vi "SwerveKinematics_ToSwerveModuleStates.vi"(9 "CenterOfRotation":T3={"X"=0.0, "Y"=1.0} {"Y" format="%14.3f"; "X" format="%14.3f"}, 10 "ChassisSpeeds":T6 {"vOmega" format="%10.3f"; "vY" format="%10.3f"; "vX" format="%10.3f"}, 11 "in SWERVE_DRIVE_KINEMATICS":T4 {"SavedModuleStates"."Angle"."SIN" format="%13.4f"; "SavedModuleStates"."Angle"."COS" format="%13.4f"; "SavedModuleStates"."Angle"."VALUE" format="%13.4f"; "PrevCoR"."Y" format="%14.3f"; "PrevCoR"."X" format="%14.3f"; "Modules"."Y" format="%14.3f"; "Modules"."X" format="%14.3f"}) -> (1 "ModuleStates":T1[](array[typedef]) {"Angle"."SIN" format="%13.4f"; "Angle"."COS" format="%13.4f"; "Angle"."VALUE" format="%13.4f"}, 3 "out SWERVE_DRIVE_KINEMATICS":T4 {"SavedModuleStates"."Angle"."SIN" format="%13.4f"; "SavedModuleStates"."Angle"."COS" format="%13.4f"; "SavedModuleStates"."Angle"."VALUE" format="%13.4f"; "PrevCoR"."Y" format="%14.3f"; "PrevCoR"."X" format="%14.3f"; "Modules"."Y" format="%14.3f"; "Modules"."X" format="%14.3f"})   [LabVIEW 2019, in "Trajectory_Library.lvlib"]
doc: "Performs inverse kinematics to return the module states from a desired chassis velocity. This method is often used to convert joystick values into module speeds and angles.\n \nThis function also supports variable centers of rotation. During normal operations, the center of rotation is usually the same as the physical center of the robot; therefore, the argument is defaulted to that use case. However, if you wish to change the center of rotation for evasive manuevers, vision alignment, or for any other use case, you can do so.\n\nIn the case that the desired chassis speeds are zero (i.e. the robot will be stationary), the previously calculated module angle will be maintained.\n \nParameters:\n - chassisSpeeds -- The desired chassis speed.\n - centerOfRotation -- The center of rotation. For example, if you set the center of rotation at one corner of the robot and provide a chassis speed that only has a dtheta component, the robot will rotate around that corner. (Meters)\n\nReturns:\n - ModuleStates - An array of data structures containing the module states. Use caution because these module states are not normalized. Sometimes, a user input may cause one of the module speeds to go above the attainable max velocity. Use the {@link #normalizeWheelSpeeds(SwerveModuleState[], double) normalizeWheelSpeeds} function to rectify this issue."
uses:
  Trajectory_Library.lvlib
  TypeDef/SWERVE_DRIVE_KINEMATICS.ctl
  <vilib>/Analysis/Matrix/Datatypes/RealMatrix.ctl
  TypeDef/TRANSLATION2D.ctl
  TypeDef/SWERVE_DRIVE_MODULE_STATE.ctl
  TypeDef/ROTATION2D.ctl
  TypeDef/CHASSIS_SPEEDS.ctl
  MatBuilder_Create.vi
  MatrixHelper_CoerceSize.vi
  <vilib>/Analysis/Matrix/Numeric/Multiply/Multiply - RM,RM.vi
  <vilib>/Analysis/Matrix/NI_Matrix.lvlib
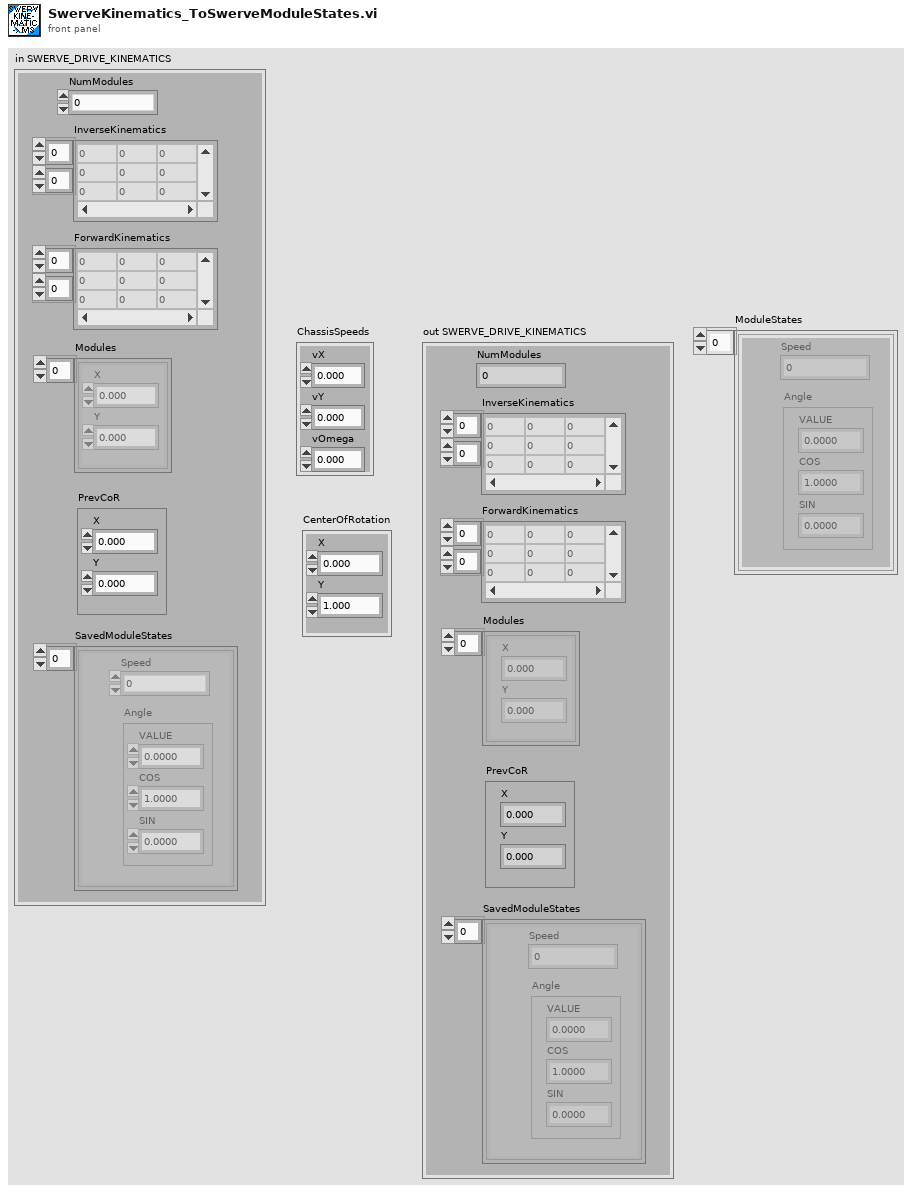
[diagram p1: front panel]
types:
  T1 = typedef "Trajectory_Library.lvlib/SWERVE_DRIVE_MODULE_STATE.ctl" = cluster{"Speed":dbl, "Angle":T2}
  T2 = typedef "Trajectory_Library.lvlib/ROTATION2D.ctl" = cluster{"VALUE":dbl, "COS":dbl, "SIN":dbl}
  T3 = typedef "Trajectory_Library.lvlib/TRANSLATION2D.ctl" = cluster{"X":dbl, "Y":dbl}
  T4 = typedef "Trajectory_Library.lvlib/SWERVE_DRIVE_KINEMATICS.ctl" = cluster{"NumModules":i32, "InverseKinematics":T5, "ForwardKinematics":T5, "Modules":T3[], "PrevCoR":T3, "SavedModuleStates":T1[]}
  T5 = typedef "NI_Matrix.lvlib/RealMatrix.ctl" = dbl[][]
  T6 = typedef "Trajectory_Library.lvlib/CHASSIS_SPEEDS.ctl" = cluster{"vX":dbl, "vY":dbl, "vOmega":dbl}
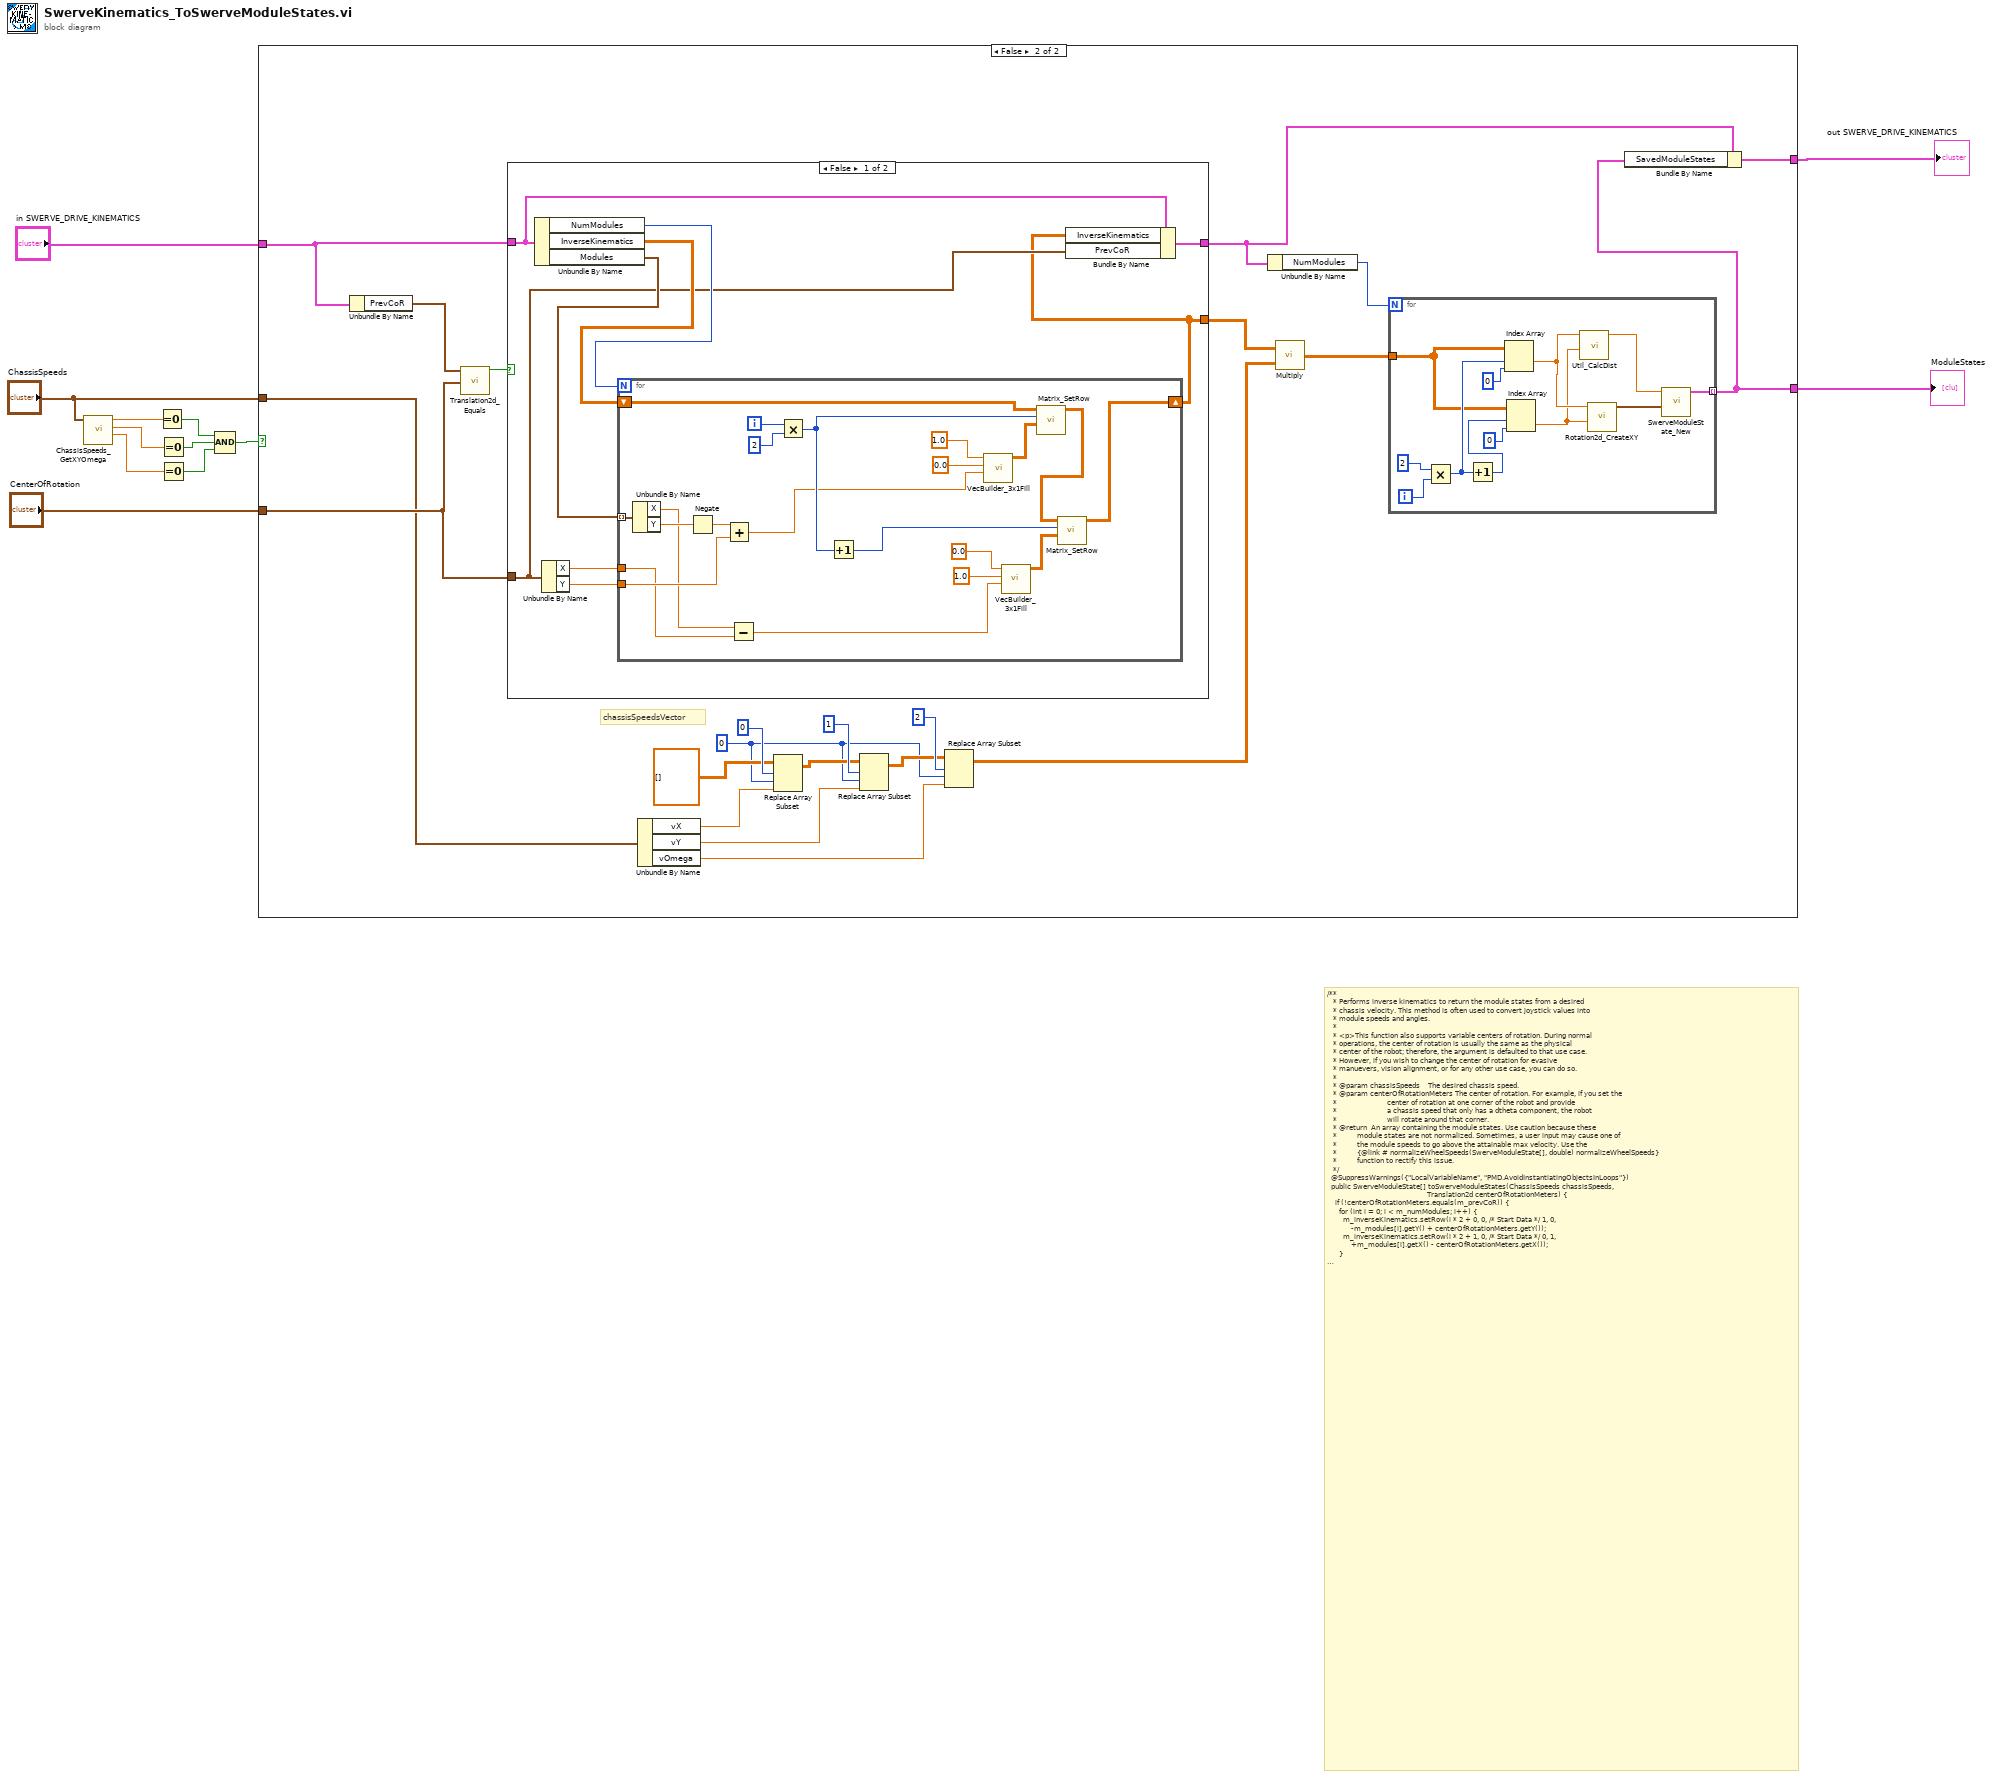
[diagram p0: block diagram]
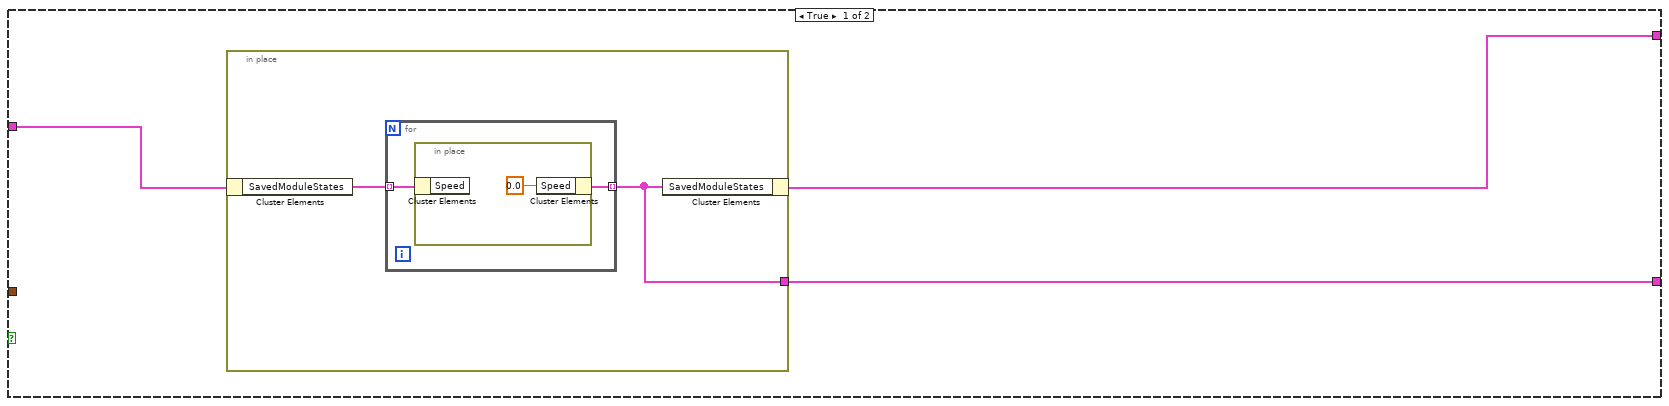
[diagram p2: hidden frame]
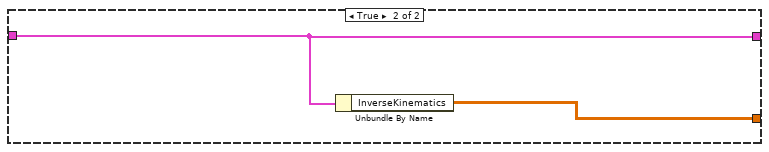
[diagram p3: hidden frame]
diagram:
  # "/**\n   * Performs inverse kinematics to return the module states from a desired\n   * chassis velocity. This method is often used to convert joystick values into\n   * module speeds and angles.\n   *\n   * <p>This function also supports variable centers of rotation. During normal\n   * operations, the center of rotation is usually the same as the physical\n   * center of the robot; therefore, the argument is defaulted to that use case.\n   * However, if you wish to change the center of rotation for evasive\n   * manuevers, vision alignment, or for any other use case, you can do so.\n   *\n   * @param chassisSpeeds    The desired chassis speed.\n   * @param centerOfRotationMeters The center of rotation. For example, if you set the\n   *                         center of rotation at one corner of the robot and provide\n   *                         a chassis speed that only has a dtheta component, the robot\n   *                         will rotate around that corner.\n   * @return  An array containing the module states. Use caution because these\n   *          module states are not normalized. Sometimes, a user input may cause one of\n   *          the module speeds to go above the attainable max velocity. Use the\n   *          {@link # normalizeWheelSpeeds(SwerveModuleState[], double) normalizeWheelSpeeds}\n   *          function to rectify this issue.\n   */\n  @SuppressWarnings({\"LocalVariableName\", \"PMD.AvoidInstantiatingObjectsInLoops\"})\n  public SwerveModuleState[] toSwerveModuleStates(ChassisSpeeds chassisSpeeds,\n                                                  Translation2d centerOfRotationMeters) {\n    if (!centerOfRotationMeters.equals(m_prevCoR)) {\n      for (int i = 0; i < m_numModules; i++) {\n        m_inverseKinematics.setRow(i * 2 + 0, 0, /* Start Data */ 1, 0,\n            -m_modules[i].getY() + centerOfRotationMeters.getY());\n        m_inverseKinematics.setRow(i * 2 + 1, 0, /* Start Data */ 0, 1,\n            +m_modules[i].getX() - centerOfRotationMeters.getX());\n      }\n      m_prevCoR = centerOfRotationMeters;\n    }\n\n    var chassisSpeedsVector = new SimpleMatrix(3, 1);\n    chassisSpeedsVector.setColumn(0, 0,\n        chassisSpeeds.vxMetersPerSecond, chassisSpeeds.vyMetersPerSecond,\n        chassisSpeeds.omegaRadiansPerSecond);\n\n    var moduleStatesMatrix = m_inverseKinematics.mult(chassisSpeedsVector);\n    SwerveModuleState[] moduleStates = new SwerveModuleState[m_numModules];\n\n    for (int i = 0; i < m_numModules; i++) {\n      double x = moduleStatesMatrix.get(i * 2, 0);\n      double y = moduleStatesMatrix.get(i * 2 + 1, 0);\n\n      double speed = Math.hypot(x, y);\n      Rotation2d angle = new Rotation2d(x, y);\n\n      moduleStates[i] = new SwerveModuleState(speed, angle);\n    }\n\n    return moduleStates;\n  }"
  n1 = call "ChassisSpeeds_GetXYOmega.vi"("CHASSIS"="ChassisSpeeds") -> ("vAngular"=w5:dbl, "vY"=w6:dbl, "vX"=w7:dbl)  [unwired: 8 in]
  n2 = Equal To 0?(x=w7) -> (x = 0?=w4:bool)
  n3 = Equal To 0?(x=w6) -> (x = 0?=w3:bool)
  n4 = Equal To 0?(x=w5) -> (x = 0?=w2:bool)
  n5 = Compound Arithmetic op=AND(w4, w3, w2) -> (w1:bool)
  n6 = case shown="False" w1 {
    tunnel: "in SWERVE_DRIVE_KINEMATICS" -> [w15 w40]
    tunnel: "CenterOfRotation" -> [_ w39]
    tunnel: "ChassisSpeeds" -> [_ w31]
    tunnel: [w13 w22] -> w10
    tunnel: [w14 w21] -> w9
    frame True {
      n7 = in-place {
        in-place-border: [w16] -> w14
        n8 = in-place-cluster #1(w15) -> ("SavedModuleStates"=w17:T1[])
        n9 = for {
          tunnel: w17 -> [w19] mode=indexing
          tunnel: [w18] -> w16 mode=indexing
          n10 = in-place {
            n11 = in-place-cluster #2(w19) -> ()  [unwired: 1 out]
            n12 = in-place-cluster #2("Speed"=0.0) -> (w18:T1)
          }
        }
        n13 = in-place-cluster #1("SavedModuleStates"=w16) -> (w13:T4)
      }
    }
    frame False {
      w32 = 0 ("disabled index (col)")
      # "chassisSpeedsVector"
      n14 = Unbundle By Name(w40) -> ("PrevCoR"=w42:T3)
      n15 = call "Translation2d_Equals.vi"("other Translation"=w39, "In Translation"=w42) -> ("Equals"=w41:bool)  [unwired: 9 in]
      n16 = case shown="False" w41 {
        tunnel: w40 -> [w57 w86]
        tunnel: [w58 w86] -> w23
        tunnel: w39 -> [w56 _]
        tunnel: [w55 w85] -> w27
        frame False {
          n17 = Unbundle By Name(w57) -> ("NumModules"=w63:i32, "InverseKinematics"=w62:T5, "Modules"=w61:T3[])
          n18 = Unbundle By Name(w56) -> ("X"=w59:dbl, "Y"=w60:dbl)
          n19 = for {
            N: w63 -> [_]
            shift-right: [w64] -> w55
            shift-left: w62 -> [w65]
            tunnel: w61 -> [w82] mode=indexing
            tunnel: w60 -> [w79]
            tunnel: w59 -> [w77]
            i -> [w84]
            n20 = Unbundle By Name(w82) -> ("X"=w78:dbl, "Y"=w81:dbl)
            n21 = Negate(x=w81) -> (-x=w80:dbl)
            n22 = Add(x=w80, y=w79) -> (x+y=w67:dbl)
            n23 = Subtract(x=w78, y=w77) -> (x-y=w66:dbl)
            n24 = Multiply(x=w84, y=2) -> (x*y=w68:i32)
            n25 = Increment(x=w68) -> (x+1=w76:i32)
            n26 = call "VecBuilder_3x1Fill.vi"("R2"=w67, "R1"=0.0, "R0"=1.0) -> ("output matrix"=w74:T5)  [unwired: 8 in]
            n27 = call "VecBuilder_3x1Fill.vi"("R2"=w66, "R1"=1.0, "R0"=0.0) -> ("output matrix"=w73:T5)  [unwired: 8 in]
            n28 = call "Matrix_SetRow.vi"("Fill Row Vector"=w74, "Row"=w68, "input matrix"=w65) -> ("output matrix"=w75:T5)  [unwired: 7 in, 1 out]
            n29 = call "Matrix_SetRow.vi"("Fill Row Vector"=w73, "Row"=w76, "input matrix"=w75) -> ("output matrix"=w64:T5)  [unwired: 7 in, 1 out]
          }
          n30 = Bundle By Name(cluster=w57, "InverseKinematics"=w55, "PrevCoR"=w56) -> (w58:T4)
        }
        frame True {
          n31 = Unbundle By Name(w86) -> ("InverseKinematics"=w85:T5)
        }
      }
      n32 = Unbundle By Name(w31) -> ("vX"=w30:dbl, "vY"=w29:dbl, "vOmega"=w28:dbl)
      n33 = Replace Array Subset(array=T5 [] ("InverseKinematics"), new element=w30, index (row)=0 ("disabled index (row)"), index (col)=w32) -> (w34:T5)
      n34 = Replace Array Subset(array=w34, new element=w29, index (row)=1 ("disabled index (row)"), index (col)=w32) -> (w33:T5)
      n35 = Replace Array Subset(array=w33, new element=w28, index (row)=2 ("disabled index (row)"), index (col)=w32) -> (w26:T5)
      n36 = Unbundle By Name(w23) -> ("NumModules"=w25:i32)
      n37 = call-poly <vilib>:"Multiply.vi"("Real Matrix B"=w26, "Real Matrix A"=w27) -> ("A * B"=w24:T5)
      n38 = for {
        N: w25 -> [_]
        tunnel: [w54] -> w21 mode=indexing
        tunnel: w24 -> [w47]
        i -> [w53]
        n39 = Multiply(x=2, y=w53) -> (x*y=w50:i32)
        n40 = Increment(x=w50) -> (x+1=w48:i32)
        n41 = Index Array(array=w47, index (row)=w50, index (col)=0) -> (element=w46:dbl)
        n42 = Index Array(array=w47, index (row)=w48, index (col)=0) -> (element=w45:dbl)
        n43 = call "Util_CalcDist.vi"("Y"=w45, "X"=w46) -> ("DIST"=w43:dbl)  [unwired: 9 in]
        n44 = call "Rotation2d_CreateXY.vi"("Y or sine"=w45, "X or  cosine"=w46) -> ("ROTATION"=w44:T2)  [unwired: 9 in]
        n45 = call "SwerveModuleState_New.vi"("ROTATION"=w44, "Speed"=w43) -> ("SWERVE_DRIVE_MODULE_STATE"=w54:T1)  [unwired: 9 in]
      }
      n46 = Bundle By Name(cluster=w23, "SavedModuleStates"=w21) -> (w22:T4)
    }
  }
  "out SWERVE_DRIVE_KINEMATICS" <- w10
  "ModuleStates" <- w9
